vi "set Marker X Position Frequency.vi"(8 "error in (no error)":errorcluster, 9 "Index":i32, 10 "X Position Frequency (Hz)":dbl, 11 "Keysight 9020A in":refnum<class "Keysight 9020A.lvclass">) -> (0 "error out":errorcluster, 3 "Keysight 9020A out":refnum<class "Keysight 9020A.lvclass">)   [LabVIEW 2023, in "Spectrum Analyzer.lvlib" / "Keysight 9020A.lvclass"]
uses:
  Keysight 9020A.lvclass
  Keysight 9020A.lvclass/Keysight 9020A.ctl
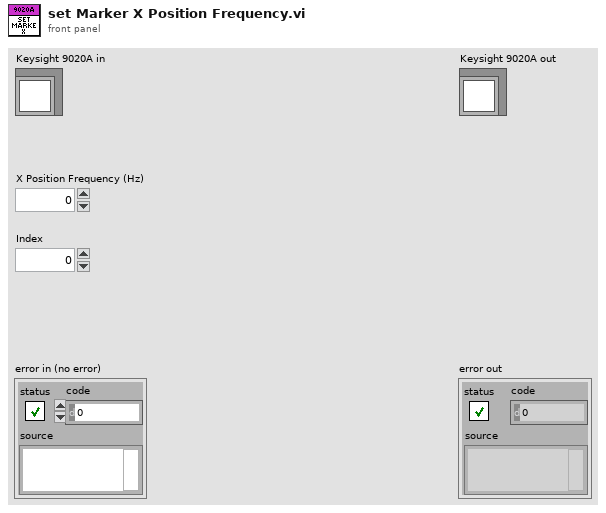
[diagram p1: front panel]
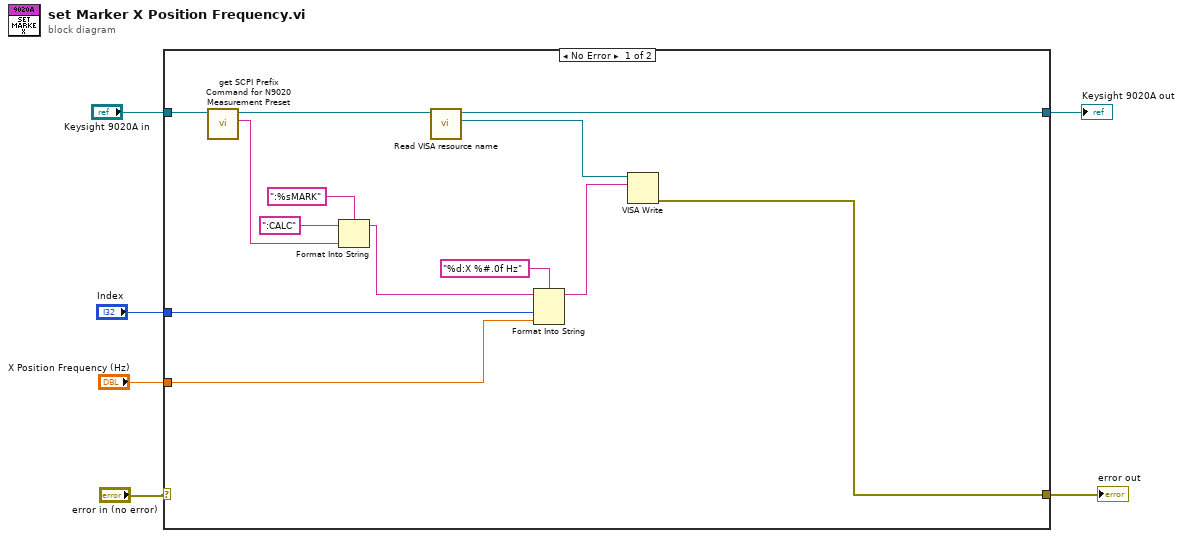
[diagram p0: block diagram]
diagram:
  n1 = case shown="No Error" "error in (no error)" {
    selector: "error in (no error)" -> [_ w20]
    tunnel: "Keysight 9020A in" -> [w14 w21]
    tunnel: [w8 w21] -> w5
    tunnel: [w16 w20] -> w3
    tunnel: "Index" -> [w17 _]
    tunnel: "X Position Frequency (Hz)" -> [w7 _]
    frame No Error {
      n2 = call "get SCPI Prefix Command for N9020 Measurement Preset.vi"("Keysight 9020A in"=w14) -> ("SCPI Prefix Command"=w11:string, "Keysight 9020A out"=w10:refnum<class "Keysight 9020A.lvclass">)  [unwired: 8 in, 1 out]
      n3 = Format Into String(format string=":%sMARK", initial string=":CALC", w11) -> (resulting string=w9:string)  [unwired: 1 in, 1 out]
      n4 = call "Read VISA resource name.vi"("Keysight 9020A in"=w10) -> ("VISA resource name"=w15:refnum<visa-resource-name>, "Keysight 9020A out"=w8:refnum<class "Keysight 9020A.lvclass">)  [unwired: 8 in, 1 out]
      n5 = Format Into String(format string="%d:X %#.0f Hz", initial string=w9, w17, w7) -> (resulting string=w19:string)  [unwired: 1 in, 1 out]
      n6 = VISA Write(VISA resource name=w15, write buffer=w19) -> (error out=w16:errorcluster)  [unwired: 1 in, 2 out]
    }
    frame Error {
    }
  }
  "error out" <- w3
  "Keysight 9020A out" <- w5
